vi "wiringPiI2CWriteReg16.vi"(8 "error in (no error)":errorcluster, 9 "value":i32, 10 "reg":i32, 11 "devID":T1) -> (0 "error out":errorcluster, 3 "return":i32)   [LabVIEW 2020, in "wiringPi.lvlib"]
doc: "<b>_______________________________________________________________</b>\n** Author: Juan José Villacorta\n** LabVIEW wrapper for C library <b> wiringPi </b>,\n** https://github.com/WiringPi/WiringPi\n<b>_______________________________________________________________</b>\n\n/*\n * wiringPiI2CWriteReg8: wiringPiI2CWriteReg16:\n * Write an 16-bit value to the given register\n *********************************************************************************\n */"
uses:
  wiringPi.lvlib
  Type Defs/I2C Device.ctl
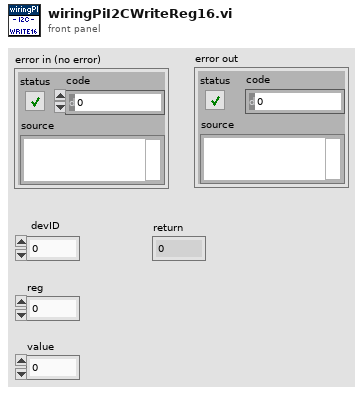
[diagram p1: front panel]
types:
  T1 = typedef "wiringPi.lvlib/I2C Device.ctl" = i32
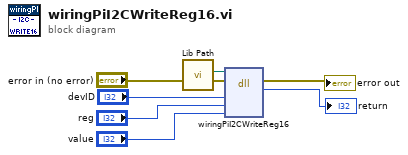
[diagram p0: block diagram]
diagram:
  n1 = call "Lib Path.vi"() -> ("path out"=w5:path)  [unwired: 11 in]
  n2 = dll-call lib="libLVwiringPI.so" fn="wiringPiI2CWriteReg16"(path in=w5, error in="error in (no error)", "fd"="devID", "reg"="reg", "value"="value") -> (error out=→"error out":errorcluster, "return type"=→"return":i32)  [unwired: 4 in, 1 out]
